vi "test1-AllChainNodesShareTheSameData.vi"(8 "error in (no error)":errorcluster, 11 "TestCase in":refnum<class "testcase-CSMChainMode.lvclass">) -> (0 "error out":errorcluster, 3 "TestCase out":refnum<class "testcase-CSMChainMode.lvclass">)   [LabVIEW 2017, in "testcase-CSMChainMode.lvclass"]
uses:
  testcase-CSMChainMode.lvclass
  src/user.lib/_NEVSTOP/Communicable State Machine(CSM)/_Support/Typedef/_CSM_MODE.ctl
  8deca385-1376-47bb-b92d-c44567c1a462.vi
  <vilib>/addons/_JKI Toolkits/VI Tester/TestCase.llb/TestCase.lvclass
  src/user.lib/_NEVSTOP/Communicable State Machine(CSM)/Communicable State Machine.lvlib
  C:/Program Files (x86)/National Instruments/LabVIEW 2017/vi.lib/addons/_JKI Toolkits/VI Tester/TestCase.llb/TestCase.lvclass
panel:
  out "LoopCount":i32
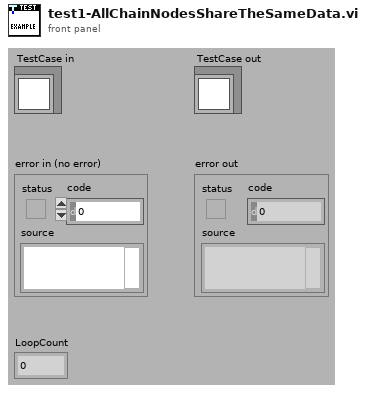
[diagram p1: front panel]
types:
  T1 = typedef "Communicable State Machine.lvlib/_CSM_MODE.ctl" = enum16{"Not Exist", "Stand Alone", "CSM", "Worker", "Worker Agent", "Chain Node", "Chain"}
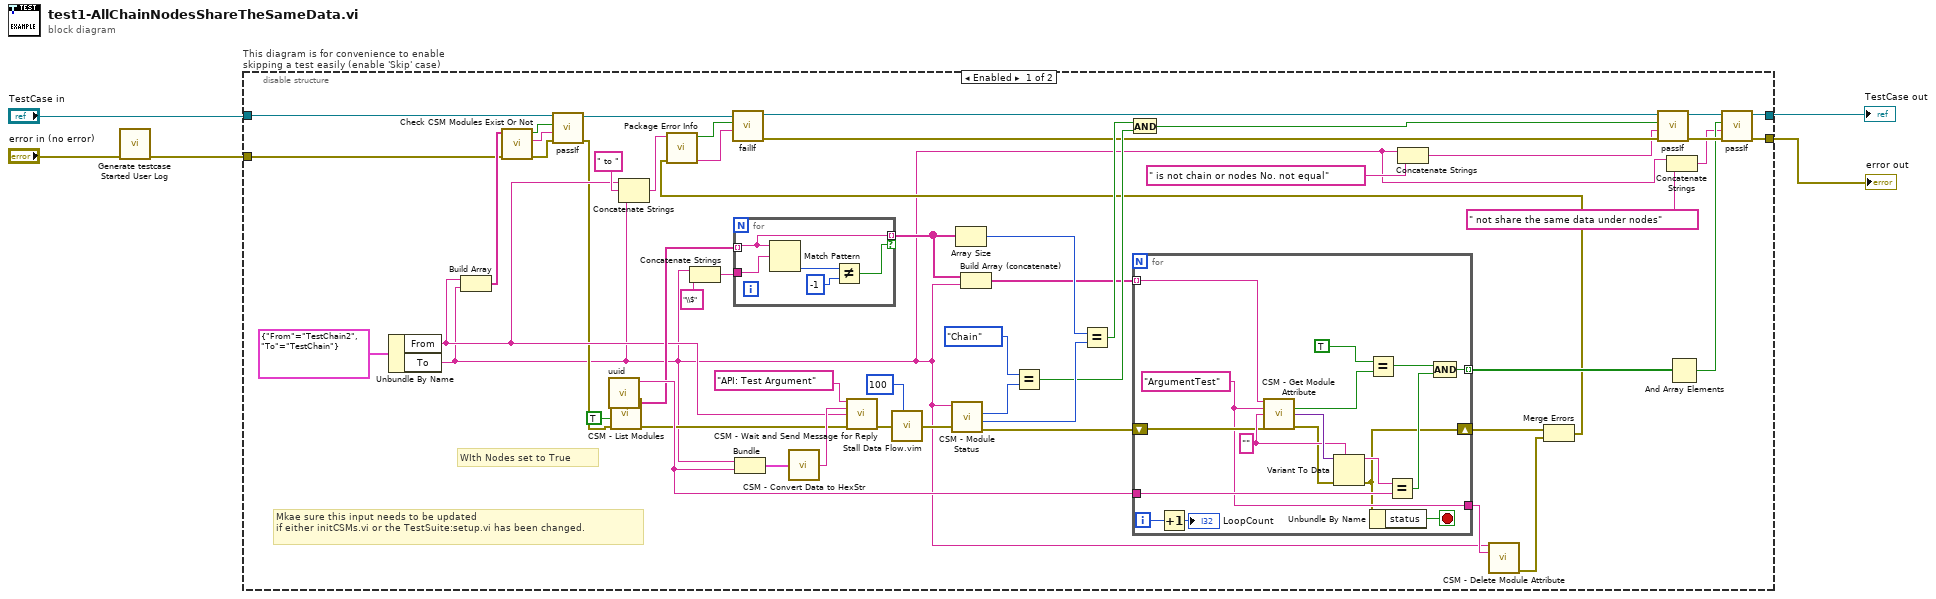
[diagram p0: block diagram]
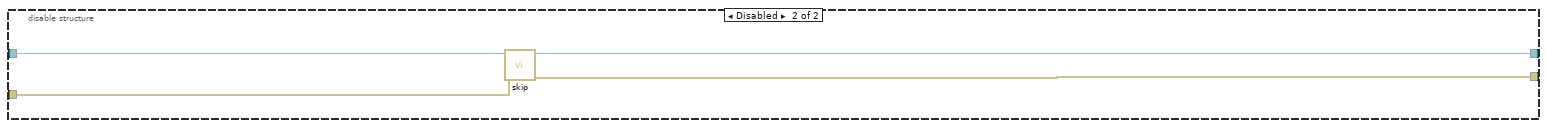
[diagram p2: hidden frame]
diagram:
  n1 = call "Generate testcase Started User Log.vi"("Error In"="error in (no error)") -> ("error out"=w1:errorcluster)  [unwired: 10 in]
  n2 = disable-structure "This diagram is for convenience to enable skipping a test easily (enable 'Skip' case)" shown="Enabled" {
    disable-tunnel: "TestCase in" -> [w14 w84]
    disable-tunnel: [w31 w82] -> w2
    disable-tunnel: [w30 w83] -> w4
    disable-tunnel: w1 -> [w22 w81]
    frame Enabled {
      # "Mkae sure this input needs to be updated \nif either initCSMs.vi or the TestSuite:setup.vi has been changed."
      # "WIth Nodes set to True"
      n3 = Unbundle By Name(cluster{"From":string, "To":string} {"From"="TestChain2", "To"="TestChain"} ("Cluster")) -> ("From"=w17:string, "To"=w7:string)
      n4 = Build Array(w17, w7) -> (w23:string[])
      n5 = call "Check CSM Modules Exist Or Not.vi"("error in"=w22, "CSM names in"=w23) -> ("error out"=w24:errorcluster, "Debug string"=w25:string, "All Modules Exist?"=w26:bool)  [unwired: 7 in]
      n6 = call-dynamic "passIf.vi"("error in (no error)"=w24, "message (\"\")"=w25, "pass"=w26, "TestCase in"=w14) -> ("error out"=w16:errorcluster, "TestCase out"=w13:refnum<class "testcase-CSMChainMode.lvclass">)  [unwired: 6 in]
      n7 = call "uuid.vi"() -> ("UUID"=w53:string)  [unwired: 11 in]
      n8 = call "CSM - List Modules.vi"("Error In"=w16, "With Nodes? (F)"=TRUE) -> ("error out"=w47:errorcluster, "Module Names"=w50:string[])  [unwired: 8 in]
      n9 = Concatenate Strings(w17, " to " ("string"), w7) -> (w18:string)
      n10 = Concatenate Strings(w7, "\\$" ("string")) -> (w28:string)
      n11 = for {
        tunnel: w50 -> [w78] mode=indexing
        tunnel: [w78] -> w39 mode=indexing if=w77
        tunnel: w28 -> [w76]
        n12 = Match Pattern(string=w78, regular expression=w76) -> (offset past match=w80:i32)  [unwired: 1 in, 3 out]
        n13 = Not Equal?(x=w80, y=-1) -> (x != y?=w77:bool)
      }
      n14 = Bundle("To"=w7, "UUID"=w53) -> (w55:cluster{"To":string, "UUID":string})  [unwired: 1 in]
      n15 = call "CSM - Convert Data to HexStr.vi"("Variant"=w55) -> ("HEX String (0-9,A-F)"=w54:string)  [unwired: 8 in]
      n16 = call "CSM - Wait and Send Message for Reply.vi"("State"="API: Test Argument", "Arguments (\"\")"=w54, "Target Module"=w17, "Error In (No Error)"=w47) -> ("error out"=w57:errorcluster)  [unwired: 8 in, 3 out]
      n17 = call "Stall Data Flow.vim"("value in"=w57, "milliseconds to wait"=u32 100) -> ("value out"=w52:errorcluster)  [unwired: 1 out]
      n18 = call "CSM - Module Status.vi"("Error In"=w52, "CSM Name"=w7) -> ("error out"=w37:errorcluster, "#Nodes"=w46:i32, "Mode"=w48:T1)  [unwired: 5 in, 2 out]
      n19 = Array Size(array=w39) -> (size(s)=w45:i32)
      n20 = Build Array (concatenate)(w39, w7) -> (w38:string[])
      n21 = Equal?(x=_CSM_MODE."Chain" ("Mode 2"), y=w48) -> (x = y?=w43:bool)
      n22 = Equal?(x=w45, y=w46) -> (x = y?=w44:bool)
      n23 = And(x=w44, y=w43) -> (x .and. y?=w42:bool)
      n24 = for {
        tunnel: w53 -> [w75]
        tunnel: w38 -> [w66] mode=indexing
        shift-right: [w60] -> w33
        shift-left: w37 -> [w65]
        tunnel: [w64] -> w36 mode=indexing
        tunnel: [w63] -> w34
        i -> [w62]
        stop <- w59 stop-if-true
        w71 = ""
        w63 = "ArgumentTest" ("Attribute")
        n25 = Increment(x=w62) -> (x+1=→"LoopCount":i32)
        n26 = call "CSM - Get Module Attribute.vi"("CSM Name"=w66, "Attribute"=w63, "Default Value (Empty Variant)"=w71, "Error In"=w65) -> ("Found"=w74:bool, "Value"=w72:variant, "error out"=w69:errorcluster)  [unwired: 7 in, 2 out]
        n27 = Variant To Data(error in=w69, type=w71, Variant=w72) -> (data=w70:string, error out=w60:errorcluster)
        n28 = Equal?(x=TRUE, y=w74) -> (x = y?=w68:bool)
        n29 = Unbundle By Name(w60) -> ("status"=w59:bool)
        n30 = Equal?(x=w70, y=w75) -> (x = y?=w67:bool)
        n31 = Compound Arithmetic op=AND(w68, w67) -> (w64:bool)
      }
      n32 = Concatenate Strings(w7, " is not chain or nodes No. not equal" ("string")) -> (w9:string)
      n33 = call "CSM - Delete Module Attribute.vi"("CSM Name"=w7, "Attribute"=w34) -> ("error out"=w32:errorcluster)  [unwired: 10 in, 3 out]
      n34 = Merge Errors(w33, w32) -> (w15:errorcluster)
      n35 = call "Package Error Info.vi"("error in"=w15, "String in"=w18) -> ("packed error info out"=w20:string, "error status"=w21:bool)  [unwired: 8 in]
      n36 = call-dynamic "failIf.vi"("message (\"\")"=w20, "fail"=w21, "TestCase in"=w13) -> ("error out"=w11:errorcluster, "TestCase out"=w12:refnum<class "testcase-CSMChainMode.lvclass">)  [unwired: 7 in]
      n37 = call-dynamic "passIf.vi"("error in (no error)"=w11, "message (\"\")"=w9, "pass"=w42, "TestCase in"=w12) -> ("error out"=w40:errorcluster, "TestCase out"=w41:refnum<class "testcase-CSMChainMode.lvclass">)  [unwired: 6 in]
      n38 = Concatenate Strings(w7, " not share the same data under nodes" ("string")) -> (w6:string)
      n39 = And Array Elements(Boolean array=w36) -> (logical AND=w35:bool)
      n40 = call-dynamic "passIf.vi"("error in (no error)"=w40, "message (\"\")"=w6, "pass"=w35, "TestCase in"=w41) -> ("error out"=w30:errorcluster, "TestCase out"=w31:refnum<class "testcase-CSMChainMode.lvclass">)  [unwired: 6 in]
    }
    frame Disabled {
      # "skip test result while test is under development"
      n41 = call <vilib>:"skip.vi"("error in (no error)"=w81, "TestCase in"=w84) -> ("error out"=w83:errorcluster, "TestCase out"=w82:refnum<class "testcase-CSMChainMode.lvclass">)  [unwired: 8 in]
    }
  }
  "error out" <- w4
  "TestCase out" <- w2
